vi "Abbreviate Item Name.vi"(9 "Config":T1, 11 "Name":string) -> (3 "Name out":string)   [LabVIEW 2020, in "VI Properties Editor.lvlib"]
doc: "Abbreviates an item name based on <B>Config</B>."
uses:
  VI Properties Editor.lvlib
  CTLs/Filter Column.ctl
  CTLs/Filter Type.ctl
  CTLs/Filter Info.ctl
  CTLs/Config.ctl
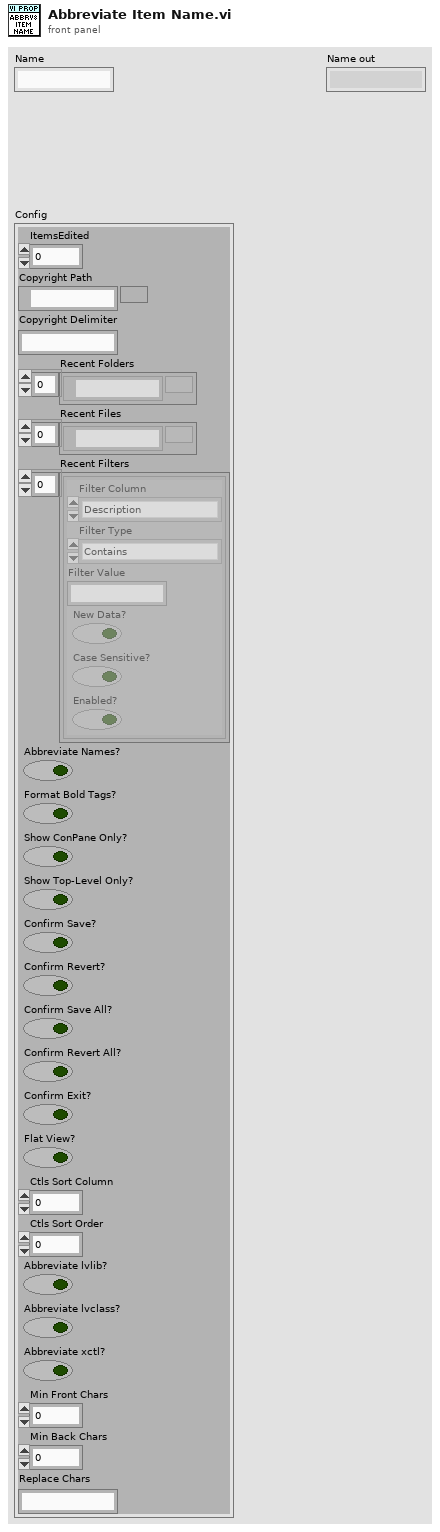
[diagram p1: front panel]
types:
  T1 = typedef "VI Properties Editor.lvlib/Config.ctl" = cluster{"ItemsEdited":u32, "Copyright Path":path, "Copyright Delimiter":string, "Recent Folders":path[], "Recent Files":path[], "Recent Filters":T2[], "Abbreviate Names?":bool, "Format Bold Tags?":bool, "Show ConPane Only?":bool, "Show Top-Level Only?":bool, "Confirm Save?":bool, "Confirm Revert?":bool, "Confirm Save All?":bool, "Confirm Revert All?":bool, "Confirm Exit?":bool, "Flat View?":bool, "Ctls Sort Column":i32, "Ctls Sort Order":i32, "Abbreviate lvlib?":bool, "Abbreviate lvclass?":bool, "Abbreviate xctl?":bool, "Min Front Chars":i32, "Min Back Chars":i32, "Replace Chars":string}
  T2 = typedef "VI Properties Editor.lvlib/Filter Info.ctl" = cluster{"Filter Column":T3, "Filter Type":T4, "Filter Value":string, "New Data?":bool, "Case Sensitive?":bool, "Enabled?":bool}
  T3 = typedef "VI Properties Editor.lvlib/Filter Column.ctl" = enum16{"Name", "Path", "Type", "Window Title", "Description", "Help Path", "Help Tag", "Custom Title?", "Reentrancy", "Inlined?", "Help URL", "Help Type", "Allow Debugging?", "Auto Error Handling?", "Run When Opened?", "Suspend When Called?", "Priority", "Preferred Exec Sytem", "Control Label", "Control Caption", "Control Description", "Control Tip Strip"}
  T4 = typedef "VI Properties Editor.lvlib/Filter Type.ctl" = enum16{"Contains", "Equals", "Starts with", "Ends with", "Is empty", "Does not contain", "Does not equal", "Is not empty"}
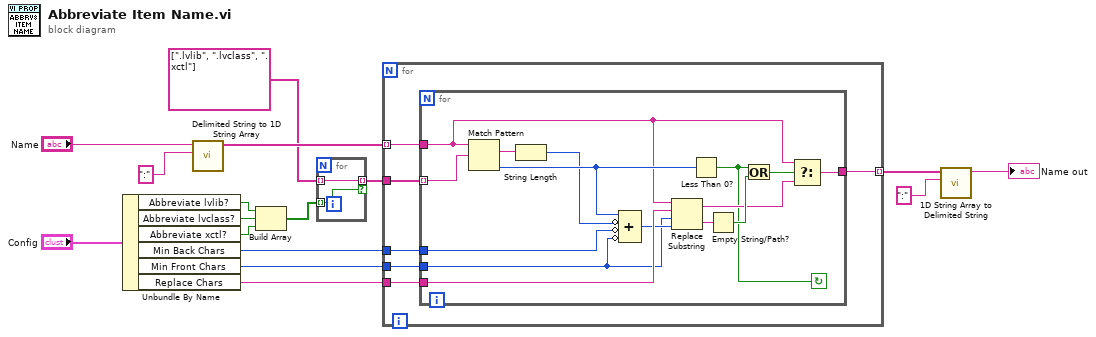
[diagram p0: block diagram]
diagram:
  n1 = Unbundle By Name("Config") -> ("Abbreviate lvlib?"=w4:bool, "Abbreviate lvclass?"=w5:bool, "Abbreviate xctl?"=w6:bool, "Min Back Chars"=w11:i32, "Min Front Chars"=w10:i32, "Replace Chars"=w9:string)
  n2 = call-poly <vilib>:"Delimited String to 1D String Array.vi"("delimiter"=":", "delimited string"="Name") -> ("string array"=w12:string[])  [unwired: 9 in]
  n3 = Build Array(w4, w5, w6) -> (w1:bool[])
  n4 = for {
    tunnel: string[] [".lvlib", ".lvclass", ".xctl"] -> [w18] mode=indexing
    tunnel: [w18] -> w2 mode=indexing if=w17
    tunnel: w1 -> [w17] mode=indexing
  }
  n5 = for {
    tunnel: w12 -> [w24] mode=indexing
    tunnel: w11 -> [w23]
    tunnel: w10 -> [w22]
    tunnel: w9 -> [w21]
    tunnel: [w20] -> w8 mode=indexing
    tunnel: w2 -> [w19]
    n6 = for {
      tunnel: w24 -> [w36]
      tunnel: w23 -> [w29]
      tunnel: w22 -> [w28]
      tunnel: w21 -> [w35]
      tunnel: [w39] -> w20
      tunnel: w19 -> [w37] mode=indexing
      stop <- w25 continue-if-true
      n7 = Match Pattern(string=w36, regular expression=w37) -> (match substring=w27:string, offset past match=w38:i32)  [unwired: 1 in, 2 out]
      n8 = String Length(string=w27) -> (length=w26:i32)
      n9 = Compound Arithmetic op=ADD(w38, invert w26, invert w29, invert w28) -> (w34:i32)
      n10 = Replace Substring(2:w34, 3:w28, 4:w35, 5:w36) -> (0:w33:string, 1:w30:string)
      n11 = Less Than 0?(x=w38) -> (x < 0?=w25:bool)
      n12 = Empty String/Path?(string/path=w33) -> (empty?=w31:bool)
      n13 = Or(x=w25, y=w31) -> (x .or. y?=w32:bool)
      n14 = Select(t=w36, s=w32, f=w30) -> (s? t:f=w39:string)
    }
  }
  n15 = call-poly <vilib>:"1D String Array to Delimited String.vi"("delimiter"=":", "string array"=w8) -> ("delimited string"=→"Name out":string)  [unwired: 9 in]
